vi "FX_Close.vi"(10 "error in (no error)":errorcluster, 11 "PLC Conn":refnum<visa-resource-name>) -> (3 "error out":errorcluster)   [LabVIEW 2026]
doc: "Use this template to build a VI to use as a subVI."
panel:
  # "ÕfÃ÷£ºêPé]Í¨Ó²º¡£ÓÐåeÕ`Ò²þÌÐÐ¡£"
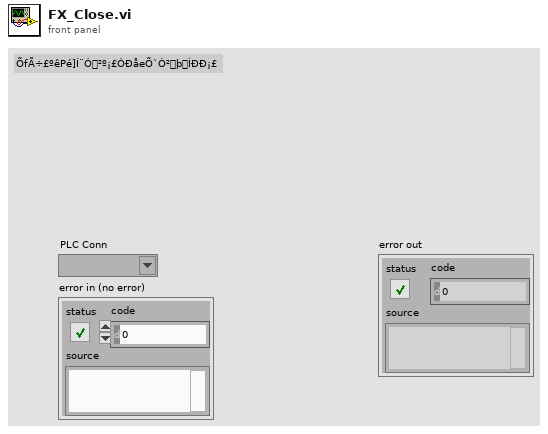
[diagram p1: front panel]
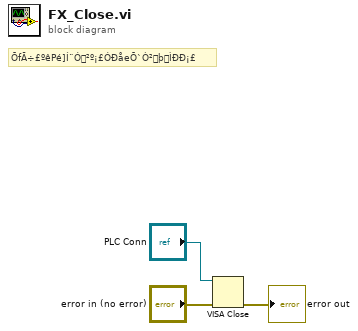
[diagram p0: block diagram]
diagram:
  # "ÕfÃ÷£ºêPé]Í¨Ó²º¡£ÓÐåeÕ`Ò²þÌÐÐ¡£"
  n1 = VISA Close(VISA resource name="PLC Conn", error in (no error)="error in (no error)") -> (error out=→"error out":errorcluster)
